vi "GetItemsByColumn.vi"(0 "Ctl Refnum In":refnum<vi>, 5 "Column Index":i32, 11 "Error In":errorcluster) -> (4 "Ctl Refnum Out":refnum<vi>, 6 "MCLB Items By Column":string[](array[string]), 15 "Error Out":errorcluster)   [LabVIEW 2019, in "Drona.lvlib"]
doc: "This VI gets MCLB items based on column index"
uses:
  Drona.lvlib
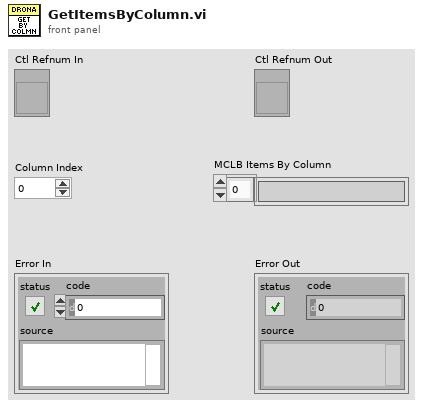
[diagram p1: front panel]
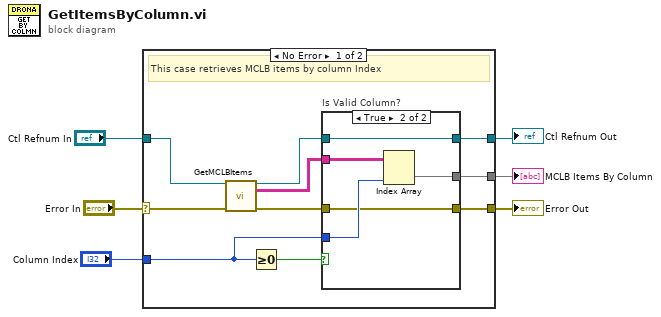
[diagram p0: block diagram]
diagram:
  n1 = case shown="No Error" "Error In" {
    selector: "Error In" -> [w16 w24]
    tunnel: "Ctl Refnum In" -> [w15 w25]
    tunnel: "Column Index" -> [w12 _]
    tunnel: [w11 _] -> w3
    tunnel: [w7 w25] -> w2
    tunnel: [w8 w24] -> w1
    frame No Error {
      # "This case retrieves MCLB items by column Index"
      n2 = call "GetMCLBItems.vi"("Ctl Refnum In"=w15, "Error In"=w16) -> ("Ctl Refnum Out"=w9:refnum<vi>, "MCLB Items"=w14:string[][], "Error Out"=w10:errorcluster)  [unwired: 11 in]
      n3 = Greater Or Equal To 0?(x=w12) -> (x >= 0?=w13:bool)
      n4 = case "Is Valid Column?" shown="True" w13 {
        tunnel: w14 -> [_ w23]
        tunnel: w12 -> [_ w22]
        tunnel: [_ w21] -> w11
        tunnel: w10 -> [w18 w20]
        tunnel: w9 -> [w17 w19]
        tunnel: [w18 w20] -> w8
        tunnel: [w17 w19] -> w7
        frame False {
        }
        frame True {
          n5 = Index Array(array=w23, index (col)=w22) -> (element=w21:string[])  [unwired: 1 in]
        }
      }
    }
    frame Error {
      # "If error, this case pass that error message only"
    }
  }
  "Error Out" <- w1
  "Ctl Refnum Out" <- w2
  "MCLB Items By Column" <- w3
